vi "Position_Feedback.vi"(8 "error in (no error)":errorcluster, 11 "Elevator in":refnum<class "Elevator.lvclass">) -> (0 "error out":errorcluster, 2 "Actual Position":dbl, 3 "Elevator out":refnum<class "Elevator.lvclass">)   [LabVIEW 2021, in "Elevator.lvclass"]
uses:
  Elevator.lvclass
  Elevator.lvclass/Elevator.ctl
  AnalogInput/AnalogInput.lvclass
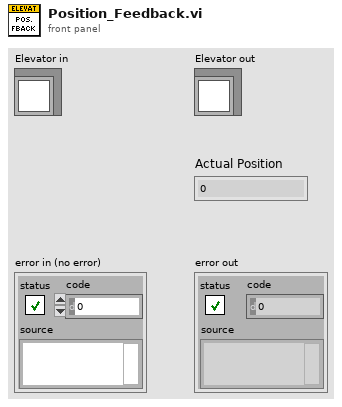
[diagram p1: front panel]
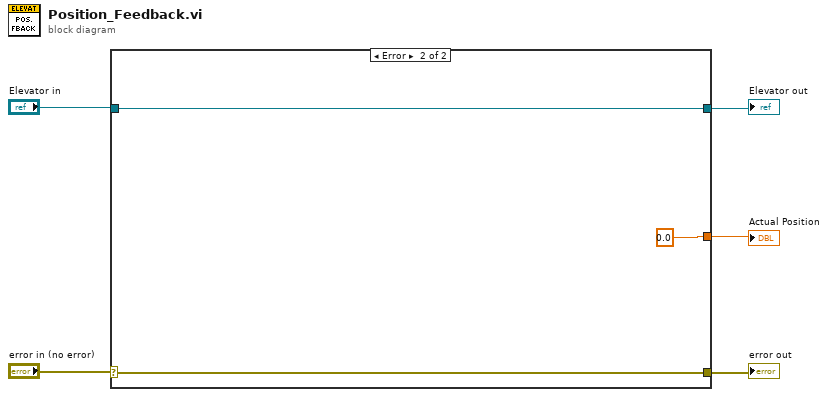
[diagram p0: block diagram]
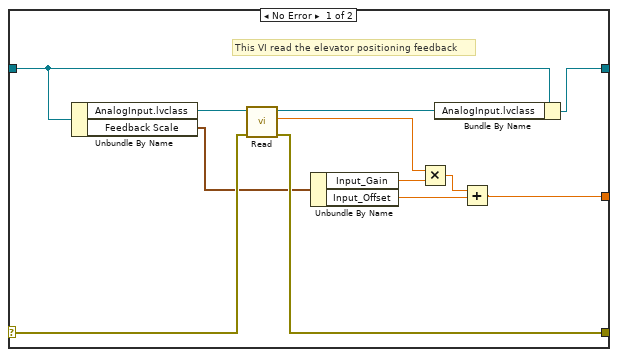
[diagram p2: hidden frame]
diagram:
  n1 = case shown="Error" "error in (no error)" {
    selector: "error in (no error)" -> [w17 w20]
    tunnel: [w15 w20] -> w3
    tunnel: [w12 w19] -> w1
    tunnel: "Elevator in" -> [w14 w19]
    tunnel: [w6 0.0 ("Data Out")] -> w2
    frame No Error {
      # "This VI read the elevator positioning feedback"
      n2 = Unbundle By Name(w14) -> ("AnalogInput.lvclass"=w16:refnum<class "AnalogInput.lvclass">, "Feedback Scale"=w11:cluster{"Input_Gain":dbl, "Input_Offset":dbl})
      n3 = call-dynamic "Read.vi"("error in (no error)"=w17, "AnalogInput in"=w16) -> ("error out"=w15:errorcluster, "Data Out"=w9:dbl, "AnalogInput out"=w13:refnum<class "AnalogInput.lvclass">)  [unwired: 7 in]
      n4 = Unbundle By Name(w11) -> ("Input_Gain"=w10:dbl, "Input_Offset"=w7:dbl)
      n5 = Multiply(x=w9, y=w10) -> (x*y=w8:dbl)
      n6 = Bundle By Name(cluster=w14, "AnalogInput.lvclass"=w13) -> (w12:refnum<class "Elevator.lvclass">)
      n7 = Add(x=w8, y=w7) -> (x+y=w6:dbl)
    }
    frame Error {
    }
  }
  "error out" <- w3
  "Elevator out" <- w1
  "Actual Position" <- w2
